vi "VIH Dialog - VI Terminals - Enum & Ring Info.vi"(8 "error in":errorcluster, 11 "Ctl Refnum":refnum<vi>) -> (0 "error out":errorcluster, 2 "EnumValDscr":T1[](array[typedef]), 3 "dup Ctl Refnum":refnum<vi>)   [LabVIEW 2014]
doc: "::: VI Helpeks :::\nCopyright (c) 2000-2026 Konstantin Shifershteyn. All rights reserved."
uses:
  _VIH HelpGen.llb/VIH HelpGen Typedef - Cluster - Enum Value Info.ctl
panel:
  # "VI Helpeks\nCopyright (c) 2012-2026 Konstantin Shifershteyn"
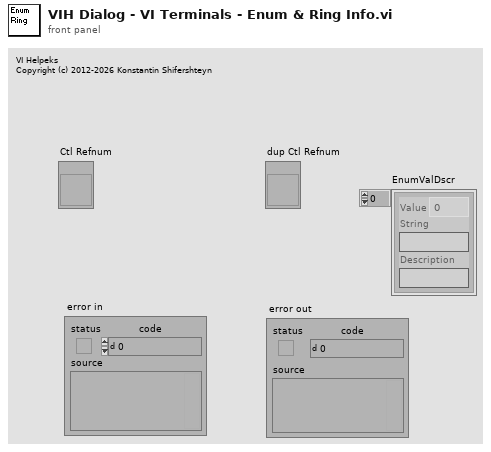
[diagram p1: front panel]
types:
  T1 = typedef "VIH HelpGen Typedef - Cluster - Enum Value Info.ctl" = cluster{"Value":ext, "String":string, "Description":string}
  T2 = typedef "LVStringsAndValuesArrayTypeDef.ctl" = cluster{"String":string, "Value":ext}[]
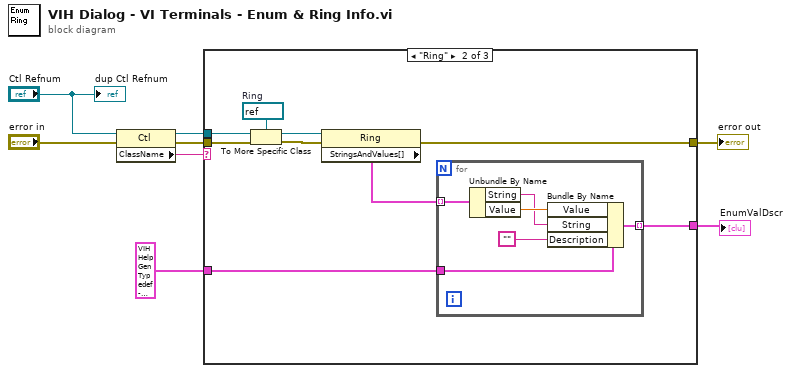
[diagram p0: block diagram]
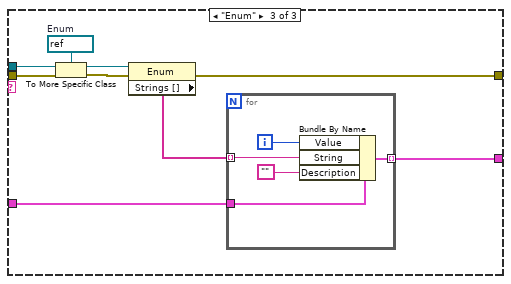
[diagram p3: hidden frame]
diagram:
  n1 = property class="Ctl"(reference="Ctl Refnum", error in="error in") -> (reference out=w5:refnum<vi>, error out=w4:errorcluster, "ClassName"=w6:string)
  n2 = case shown="\"Ring\"" w6 {
    tunnel: w5 -> [_ w18 w33]
    tunnel: w4 -> [w9 w17 w32]
    tunnel: T1 {"Value"=0.0, "String"="", "Description"=""} ("Enum Value") -> [_ w13 w25]
    tunnel: [_ w12 w28] -> w2
    tunnel: [w9 w11 w27] -> w1
    frame Default {
    }
    frame "Ring" {
      w16 = refnum<vi> refnum  # Ring
      n3 = To More Specific Class(target class=w16, reference=w18, error in=w17) -> (specific class reference=w15:refnum<vi>, error out=w14:errorcluster)
      n4 = property class="Ring"(reference=w15, error in=w14) -> (error out=w11:errorcluster, "StringsAndValues[]"=w10:T2)  [unwired: 1 out]
      n5 = for {
        tunnel: w10 -> [w24] mode=indexing
        tunnel: w13 -> [w23]
        tunnel: [w19] -> w12 mode=indexing
        n6 = Unbundle By Name(w24) -> ("String"=w21:string, "Value"=w22:ext)
        n7 = Bundle By Name(cluster=w23, "Value"=w22, "String"=w21, "Description"="") -> (w19:T1)
      }
    }
    frame "Enum" {
      w31 = refnum<vi> refnum  # Enum
      n8 = To More Specific Class(target class=w31, reference=w33, error in=w32) -> (specific class reference=w30:refnum<vi>, error out=w29:errorcluster)
      n9 = property class="Enum"(reference=w30, error in=w29) -> (error out=w27:errorcluster, "Strings []"=w26:string[])  [unwired: 1 out]
      n10 = for {
        tunnel: w25 -> [w38]
        tunnel: [w36] -> w28 mode=indexing
        tunnel: w26 -> [w35] mode=indexing
        i -> [w34]
        n11 = Bundle By Name(cluster=w38, "Value"=w34, "String"=w35, "Description"="") -> (w36:T1)
      }
    }
  }
  "error out" <- w1
  "EnumValDscr" <- w2
  "dup Ctl Refnum" <- "Ctl Refnum"
